vi "plotting_subvi__f60fe1654c.vi"(6 "commanded strain":dbl[](array[numeric]), 9 "real strain (-)":dbl[](array[numeric]), 10 "iteration":dbl, 11 "current":dbl[](array[numeric])) -> (2 "Mixed Signal Graph":dynamicdata(graph) caption="Commanded and Actual Strain vs Current", 3 "Lissajou":cluster{dbl[], dbl[]}(graph))   [LabVIEW 2023]
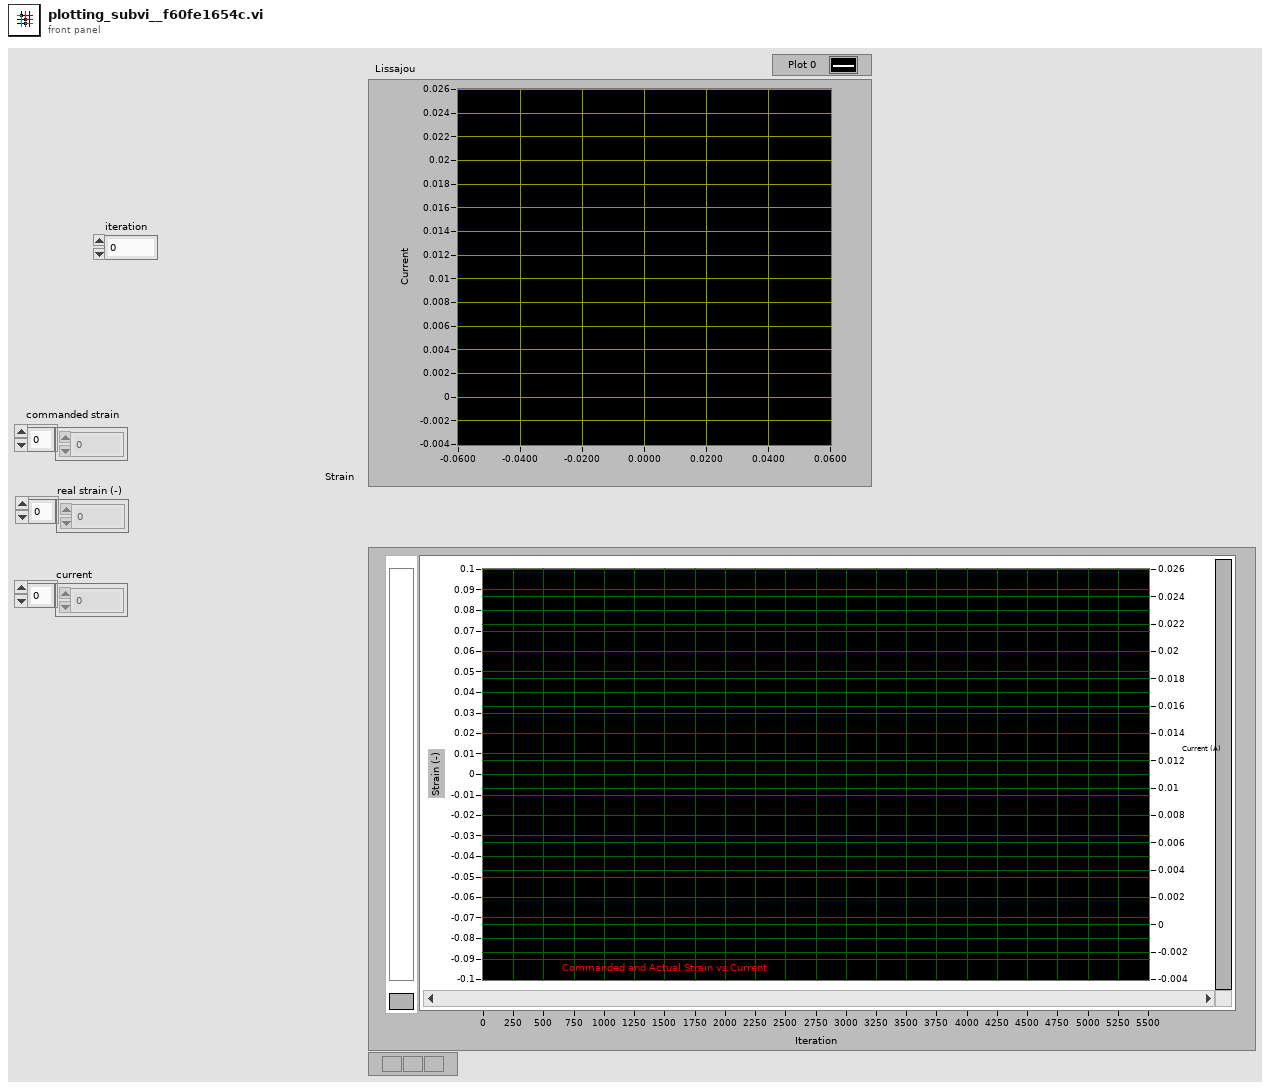
[diagram p1: front panel]
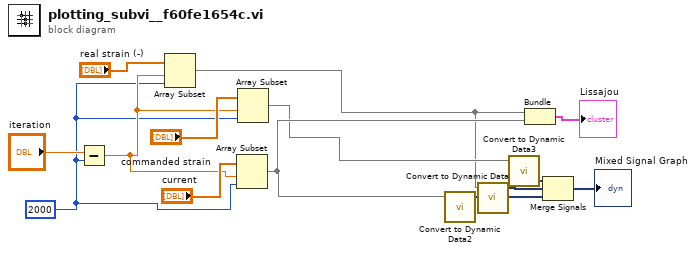
[diagram p0: block diagram]
diagram:
  w1 = 2000 ("length")
  n1 = Subtract(x="iteration", y=w1) -> (x-y=w2:dbl)
  n2 = Array Subset(array="real strain (-)", index=w2, length=w1) -> (w4:dbl[])
  n3 = Array Subset(array="current", index=w2, length=w1) -> (w9:dbl[])
  n4 = Array Subset(array="commanded strain", index=w2, length=w1) -> (w6:dbl[])
  n5 = call "Convert to Dynamic Data2"("Array"=w9) -> ("Dynamic Data Type"=w12:dynamicdata)  [unwired: 3 in]
  n6 = call "Convert to Dynamic Data"("Array"=w4) -> ("Dynamic Data Type"=w11:dynamicdata)  [unwired: 3 in]
  n7 = call "Convert to Dynamic Data3"("Array"=w6) -> ("Dynamic Data Type"=w14:dynamicdata)  [unwired: 3 in]
  n8 = Bundle(w4, w9) -> (→"Lissajou":cluster{dbl[], dbl[]})  [unwired: 1 in]
  n9 = Merge Signals(w14, w11, w12) -> (→"Mixed Signal Graph":dynamicdata)
